vi "[ex ce] Data acquisition, logging & control.vi"() -> ()   [LabVIEW 2021]
doc: "<B>Laboratory Application Example</B>\n\nThis VI demonstrates the following CalcExpress' features that can be used to build data logging, monitoring and control applications:\n-- using a CSE script to implement a control algorithm\n-- using aliases as test parameter tags\n-- automatic maintenance of variable histories\n-- storing variable histories in log files\n-- etc.\n\nThe VI is an engine of an example application that controls some virtual laboratory setup. It simulates measurement of test parameters and controlling the setup. CSE script is used to process input data, calculate an estimated parameter and determine a control value. The VI configures VarMan to automatically store history of required parameters (both measured and estimated). In addition, VI writes parameter values to log files. In order to view historical trends of parameters, use '[ex ce] Data Viewer.vi'.\n\n::: CalcExpress Toolkit :::\nCopyright (c) 2000-2026 Konstantin Shifershteyn. All rights reserved."
panel:
  in  "Delete Logfiles at end":bool=TRUE
  in  "script selector":u16(ring) caption="Script selector (select a script to execute before run the VI)" items=["Execute a simple test (Script 1)", "Execute test sequence (Script 2)"]
  in  "finalization method":bool=TRUE
  in  "script 2":string="/* Definition of local variables */\ndbl(\"Test\", 0); dbl(\"state\", 0); dbl(\"Ctrl\", Control);\n\n/* Definition of test sequence parameters */\nLevel_HI = vector(5.0, 7.0, 8.0, 8.5); //high levels\nLevel_LO = vector(2.0, 4.0, 3.0, 1.5); //low levels\nCtrl_HI  = vector(4.0, 5.0, 5.0, 6.0); //controls if high\nCtrl_LO  = vector(2.0, 0.5, 0.2, 0.0); //controls if low\n\n/* Get test parameter values from analog input data */\nPar1 = AIData[0];\nPar2 = AIData[1];\n\n/* Calculate an estimated parameter */\nEstPar = sqrt(2*Par1 * (Par2 + 1));\n\nif (state == 0) {\n  state = 1;\n  msg = sform(\"Conditioning to start Test %d\", Test+1);\n}\nif (state == 1) { //coerce Par1 to an initial value\n  if (Par1 < Level_LO[Test]) { //if good value\n    state = 2;    //next state\n    msg = sform(\"Test %d initial condition is met\", Test+1);\n  }\n  if (Par1 <= Level_LO[Test]) Ctrl = Ctrl_LO[Test];\n  else                        Ctrl = Ctrl_HI[Test];\n}\nelse if (state == 2) { //waiting for a start test condition\n  if (Par1 > Level_LO[Test] * 1.00) {\n    state = 3;    //next state\n    msg = sform(\"Test %d is running\", Test+1);\n  }\n  Ctrl = Ctrl_LO[Test];\n}\nelse if (state == 3) {   // test is running\n  if (Par1 < Level_LO[Test]) {   //test completed?\n    state = 0;\n    msg  = sform(\"Test %d is completed\", Test+1);\n    Test = (Test+1)%size(Level_LO);  //next test index\n  }\n  else\n    if (Par1 >= Level_HI[Test])  Ctrl = Ctrl_HI[Test];\n}\nelse\n  msg = sform(\"Unknown state value: %d\", state);\n\nControl = Ctrl; /*causes updating a history of Control */\n\n/* Prepare data for analog output */\nif (size(AOData) < 8) AOData = vectorn(0,8);\nAOData[0] = Control;\n" caption="Script 2 executes a sequence of four tests with conditioning to start a test"
  out "info":string="This VI demonstrates the following CalcExpress features that can be used to build data logging, monitoring and control applications:\n- using a script to implement a control algorithm\n- using aliases as test parameter tags\n- automatical maintenance of variable histories\n- storing variable histories to log files\n- etc.\nThe VI is an engine of an example application that controls some virtual laboratory setup. It simulates measurement of test parameters and controlling the setup. CSE script is used to process input data, calculate an estimated parameter and determine a control value. The VI configures VarMan to automatically store history of required parameters (both measured and estimated). In addition, VI stores parameter values to log files. In order to view historical trends of parameters, use '[ex ce] Data Viewer.vi'.\n"
  in  "save period, sec":i32=5
  out "time of last saving":dbl format="%<%H:%M:%S\n%d/%m/%Y>T"
  out "log error":bool
  in  "Write Logfiles":bool=TRUE
  out "Datalog Folder":path
  in  "initial variable definitions":T1(array[cluster])=[{"var"="AIData", "tag"="", "type"=enum."1D Array of DBL", "history len"=0}, {"var"="AOData", "tag"="", "type"=enum."1D Array of DBL", "history len"=0}, {"var"="Par1", "tag"="Test Parameter 1", "type"=enum."DBL Number", "history len"=600}, {"var"="Par2", "tag"="Test Parameter 2", "type"=enum."DBL Number", "history len"=600}, {"var"="EstPar", "tag"="Estimated Parameter", "type"=enum."DBL Number", "history len"=600}, {"var"="Control", "tag"="Control Signal", "type"=enum."DBL Number", "history len"=600}, {"var"="msg", "tag"="Message", "type"=enum."String", "history len"=50}]
  out "proc error":errorcluster
  in  "stop":bool
  in  "script 1":string="/* Get test parameter values from analog input data */\nPar1 = AIData[0]; Par2 = AIData[1];\n\n/* Calculate an estimated parameter */\nEstPar = mean(Par1, Par2);\n\n/* Determine control value */\nif      (Par1 <= 3) Control = 0;\nelse if (Par1 >= 8) Control = 4;\nelse                Control = Control; /*update history*/\n\n/* Prepare data for analog output */\nif (size(AOData) < 8) AOData = vectorn(0,8);\nAOData[0] = Control;\n" caption="Script 1 executes a simple test"
  # "*) A variable history is updated when a value is written to the variable"
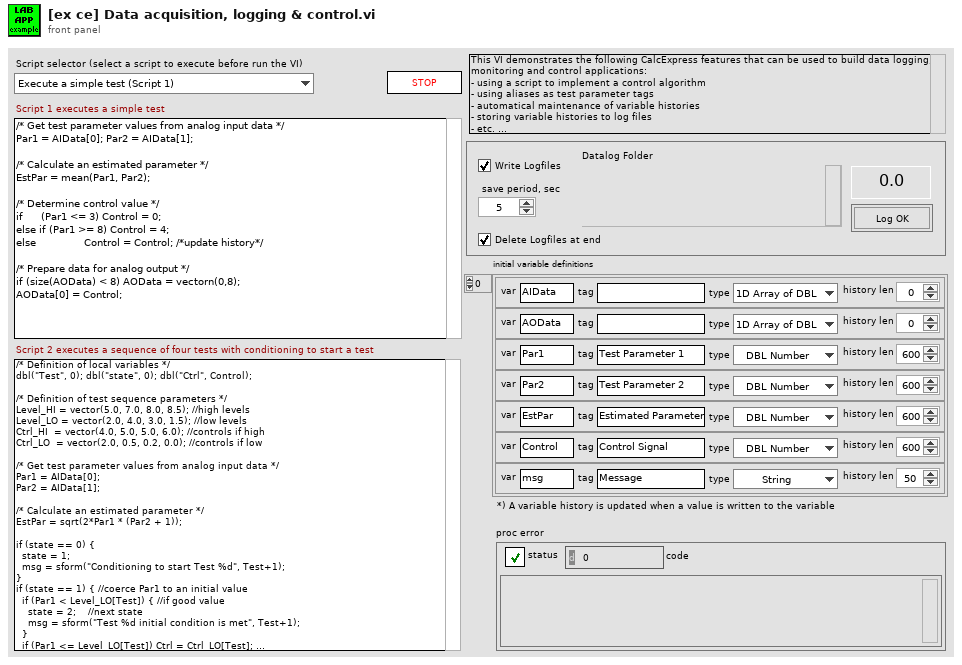
[diagram p1: front panel]
types:
  T1 = cluster{"var":string, "tag":string, "type":enum32{"String", "DBL Number", "identifier", "1D Array of DBL", "2D Array of DBL", "CDB Number", "1D Array of CDB", "2D Array of CDB", "1D Array of String", "2D Array of String", "Unknown data type"}, "history len":i32}[]
  T2 = typedef "VarMan Variable Context Handle.ctl" = i32
  T3 = enum16{"create", "destroy", "set value", "get value"}
  T4 = typedef "CSE Instance RefNum.ctl" = refnum<k1>
  T5 = enum32{"nothing", "reset", "assign name", "get name", "get handle"}
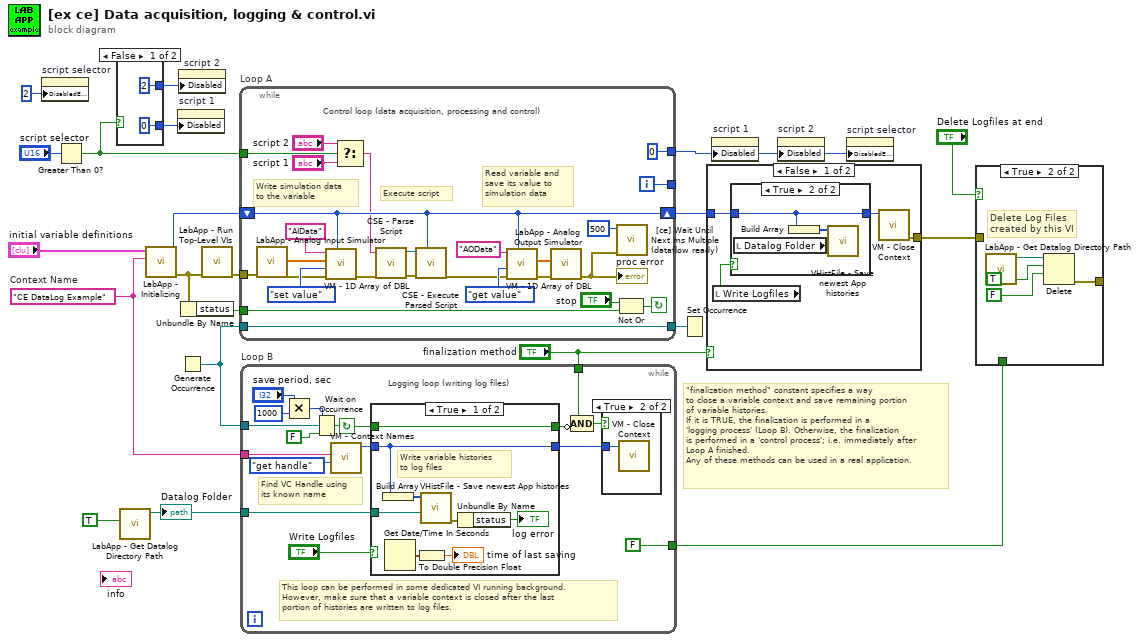
[diagram p0: block diagram]
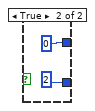
[diagram p5: hidden frame]
diagram:
  w18 = "CE DataLog Example"  # Context Name
  # "\"finalization method\" constant specifies a way\nto close a variable context and save remaining portion\nof variable histories.\nIf it is TRUE, the finalization is performed in a\n'logging process' (Loop B). Otherwise, the finalization\nis performed in a 'control process'; i.e. immediately after\nLoop A finished.\nAny of these methods can be used in a real application."
  n1 = property on="script selector" class="Ring (strict)"("DisabledEnum"=u8 2 ("Disabled")) -> ()  [unwired: 2 in, 2 out]
  n2 = Greater Than 0?(x="script selector") -> (x > 0?=w8:bool)
  n3 = case shown="False" w8 {
    tunnel: [u8 2 ("Disabled") u8 0 ("Disabled")] -> w11
    tunnel: [u8 0 ("Disabled") u8 2 ("Disabled")] -> w12
    frame False {
    }
    frame True {
    }
  }
  n4 = call "LabApp - Get Datalog Directory Path.vi"("Ena Create (F)"=TRUE) -> ("path"=w5:path)  [unwired: 9 in, 1 out]
  "Datalog Folder" <- w5
  n5 = call "LabApp - Initializing.vi"("Context Name"=w18, "variable definitions"="initial variable definitions") -> ("error out"=w15:errorcluster, "VC Handle out"=w21:T2)  [unwired: 6 in]
  n6 = property on="script 1" class="Str"("Disabled"=w12) -> ()  [unwired: 2 in, 2 out]
  n7 = Generate Occurrence() -> (w10:refnum<k4>)
  n8 = property on="script 2" class="Str"("Disabled"=w11) -> ()  [unwired: 2 in, 2 out]
  n9 = Unbundle By Name(w15) -> ("status"=w16:bool)
  n10 = call "LabApp - Run Top-Level VIs.vi"("error in (no error)"=w15) -> ("error out"=w17:errorcluster)  [unwired: 8 in]
  n11 = while "Loop A" {
    tunnel: [u8 0] -> w7
    tunnel: w8 -> [w34]
    tunnel: w16 -> [w37]
    tunnel: w10 -> [w43]
    tunnel: [w43] -> w20
    tunnel: w17 -> [w44]
    shift-left: w21 -> [w27]
    shift-right: [w27] -> w14
    tunnel: [w30] -> _
    i -> [w30]
    stop <- w38 continue-if-true
    # "Read variable and\nsave its value to\nsimulation data"
    # "Write simulation data\nto the variable"
    # "Execute script"
    # "Control loop (data acquisition, processing and control)"
    n12 = call "LabApp - Analog Input Simulator.vi"("error in"=w44) -> ("error out"=w49:errorcluster, "Data Out"=w48:dbl[])  [unwired: 7 in]
    n13 = call "VM - 1D Array of DBL.vi"("VC Handle"=w27, "error in"=w49, "cmd"=T3."set value", "value in"=w48, "name_spec"="AIData") -> ("error out"=w29:errorcluster)  [unwired: 1 in, 5 out]
    n14 = Select(t="script 2", s=w34, f="script 1") -> (s? t:f=w26:string)
    n15 = call "CSE - Parse Script.vi"("error in"=w29, "Script"=w26) -> ("error out"=w31:errorcluster, "CSE RefNum"=w32:T4)  [unwired: 5 in, 3 out]
    n16 = call "CSE - Execute Parsed Script.vi"("VC Handle"=w27, "error in"=w31, "CSE RefNum"=w32) -> ("error out"=w28:errorcluster)  [unwired: 4 in, 4 out]
    n17 = call "VM - 1D Array of DBL.vi"("VC Handle"=w27, "error in"=w28, "cmd"=T3."get value", "name_spec"="AOData") -> ("error out"=w42:errorcluster, "value out"=w41:dbl[])  [unwired: 2 in, 4 out]
    n18 = call "LabApp - Analog Output Simulator.vi"("error in"=w42, "Data In"=w41) -> ("error out"=w40:errorcluster)  [unwired: 7 in]
    "proc error" <- w40
    n19 = Not Or(1:w37, 2:"stop") -> (0:w38:bool)
    n20 = call "[ce] Wait Until Next ms Multiple (dataflow ready).vi"("error in"=w40, "millisecond multiple"=u32 500 ("milliseconds to wait")) -> ()  [unwired: 3 in, 5 out]
  }
  n21 = while "Loop B" {
    tunnel: "finalization method" -> [w54]
    tunnel: w10 -> [w67]
    tunnel: w18 -> [w63]
    tunnel: w5 -> [w53]
    tunnel: [FALSE] -> w1
    stop <- w66 continue-if-true
    # "Find VC Handle using\nits known name"
    # "This loop can be performed in some dedicated VI running background.\nHowever, make sure that a variable context is closed after the last\nportion of histories are written to log files."
    # "Logging loop (writing log files)"
    n22 = Multiply(x="save period, sec", y=1000) -> (x*y=w59:i32)
    n23 = Wait on Occurrence(1:FALSE ("ignore previous (T)"), 2:w67, 3:w59) -> (0:w66:bool)
    n24 = call "VM - Context Names.vi"("action"=T5."get handle", "VC Name"=w63) -> ("VC Handle out"=w58:T2)  [unwired: 4 in, 3 out]
    n25 = case shown="True" "Write Logfiles" {
      tunnel: w66 -> [w70 w77]
      tunnel: w58 -> [w71 w78]
      tunnel: w53 -> [w74 _]
      tunnel: [w71 w78] -> w55
      tunnel: [w70 w77] -> w57
      frame True {
        # "Write variable histories\nto log files"
        n26 = Build Array(w71) -> (w75:T2[])
        n27 = Get Date/Time In Seconds() -> (seconds since 1Jan1904=w69:timestamp)
        n28 = To Double Precision Float(number=w69) -> (double precision float=→"time of last saving":dbl)
        n29 = call "VHistFile - Save newest App histories.vi"("log directory"=w74, "app vc handles"=w75) -> ("error out"=w73:errorcluster)  [unwired: 9 in]
        n30 = Unbundle By Name(w73) -> ("status"=→"log error":bool)
      }
      frame False {
      }
    }
    n31 = Compound Arithmetic op=AND(w54, invert w57) -> (w56:bool)
    n32 = case shown="True" w56 {
      tunnel: w55 -> [_ w68]
      frame False {
      }
      frame True {
        n33 = call "VM - Close Context.vi"("VC Handle"=w68) -> ()  [unwired: 9 in, 2 out]
      }
    }
  }
  n34 = Set Occurrence(w20) -> ()
  n35 = case shown="False" "finalization method" {
    tunnel: w14 -> [w82 _]
    tunnel: [w79 _] -> w2
    frame False {
      n36 = local read "Write Logfiles"() -> (w80:bool)
      n37 = case shown="True" w80 {
        tunnel: w82 -> [w83 w84]
        tunnel: [w83 w84] -> w81
        frame False {
        }
        frame True {
          n38 = local read "Datalog Folder"() -> (w85:path)
          n39 = Build Array(w84) -> (w86:T2[])
          n40 = call "VHistFile - Save newest App histories.vi"("log directory"=w85, "app vc handles"=w86) -> ()  [unwired: 9 in, 1 out]
        }
      }
      n41 = call "VM - Close Context.vi"("VC Handle"=w81) -> ("error out"=w79:errorcluster)  [unwired: 9 in, 1 out]
    }
    frame True {
    }
  }
  n42 = property on="script 1" class="Str"("Disabled"=w7) -> ()  [unwired: 2 in, 2 out]
  n43 = property on="script 2" class="Str"("Disabled"=w7) -> ()  [unwired: 2 in, 2 out]
  n44 = property on="script selector" class="Ring (strict)"("DisabledEnum"=w7) -> ()  [unwired: 2 in, 2 out]
  n45 = case shown="True" "Delete Logfiles at end" {
    tunnel: w2 -> [_ _]
    tunnel: [_ w87] -> _
    tunnel: w1 -> [_ _]
    frame False {
    }
    frame True {
      # "Delete Log Files\ncreated by this VI"
      n46 = call "LabApp - Get Datalog Directory Path.vi"() -> ("path"=w88:path)  [unwired: 10 in, 1 out]
      n47 = Delete(path (use dialog)=w88, entire hierarchy (F)=TRUE, confirm (F)=FALSE) -> (error out=w87:errorcluster)  [unwired: 2 in, 2 out]
    }
  }
